vi "RDC-water-save_files.vi"(7 "Path":path=path "C:/projects/Universitet/Master/data/watertemp/convert water/water", 9 "temp":dbl, 10 "Common Format":T1) -> ()   [LabVIEW 2020, in "RDC-Reflection_Data_Computation.lvlib"]
doc: "Saves a Common Format cluster as a common-format file in the given folder, with the temperature in the file name."
uses:
  RDC-Reflection_Data_Computation.lvlib
  Reflector/RFH-common_data_format.ctl
  Reflector/RFH-Reflection_File_Handler.lvlib
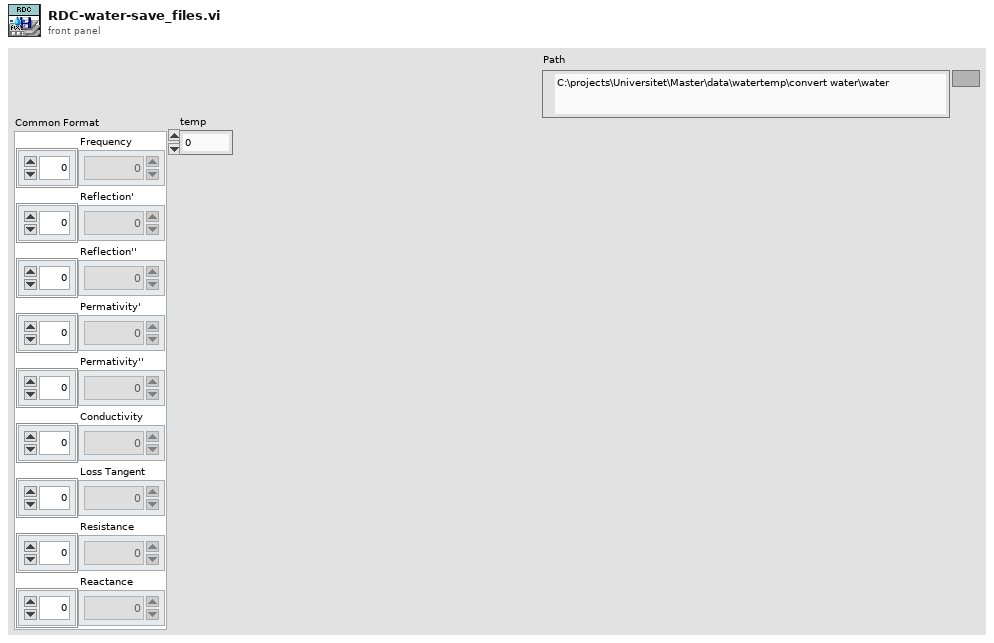
[diagram p1: front panel]
types:
  T1 = typedef "RFH-Reflection_File_Handler.lvlib/RFH-common_data_format.ctl" = cluster{"Frequency":dbl[], "Reflection'":dbl[], "Reflection''":dbl[], "Permativity'":dbl[], "Permativity''":dbl[], "Conductivity":dbl[], "Loss Tangent":dbl[], "Resistance":dbl[], "Reactance":dbl[]}
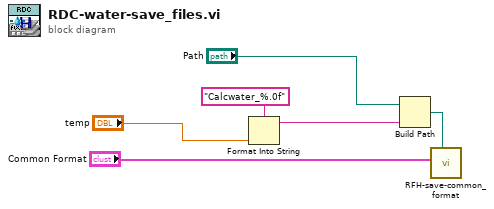
[diagram p0: block diagram]
diagram:
  n1 = Format Into String(format string="Calcwater_%.0f", "temp") -> (resulting string=w5:string)  [unwired: 2 in, 1 out]
  n2 = Build Path(base path="Path", name or relative path=w5) -> (appended path=w4:path)
  n3 = call "RFH-save-common_format.vi"("file path (use dialog)"=w4, "Common Format"="Common Format") -> ()  [unwired: 9 in, 1 out]
